vi "TwoButtonDialogWithEvent.vi"(0 "message":string, 2 "File dialog event":T1, 5 "T button name (\"OK\")":string, 7 "F button name (\"Cancel\")":string) -> ()   [LabVIEW 2025]
uses:
  FileDialogResult.ctl
  FileDialogEvent.ctl
panel:
  in  "File dialog result":T2
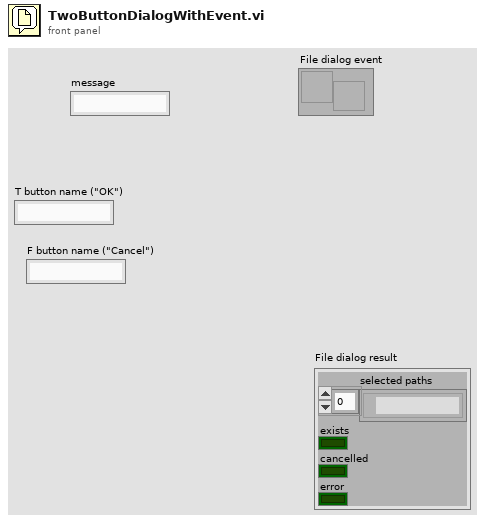
[diagram p1: front panel]
types:
  T1 = typedef "FileDialogEvent.ctl" = refnum<user-event>
  T2 = typedef "FileDialogResult.ctl" = cluster{"selected paths":path[], "exists":bool, "cancelled":bool, "error":bool}
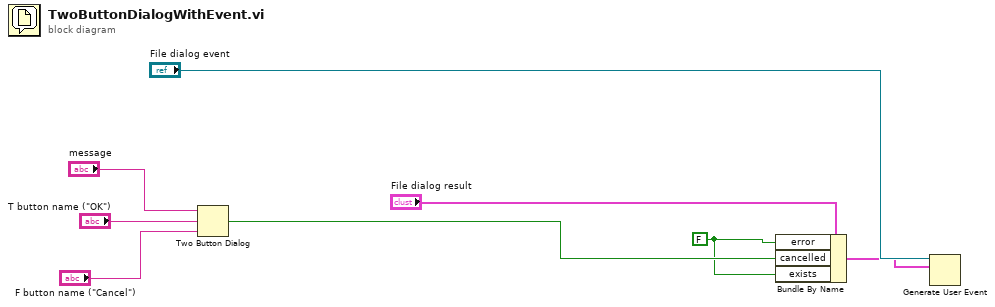
[diagram p0: block diagram]
diagram:
  w3 = FALSE ("error")
  n1 = Two Button Dialog(message="message", 1:"F button name (\"Cancel\")", 2:"T button name (\"OK\")") -> (T button?=w4:bool)
  n2 = Bundle By Name(cluster="File dialog result", "error"=w3, "cancelled"=w4, "exists"=w3) -> (w6:T2)
  n3 = Generate User Event(user event="File dialog event", event data cluster=w6) -> ()  [unwired: 2 in, 2 out]
